vi "Read Scalar Boolean.vi"(8 "error in (no error)":errorcluster, 11 "pointer in":u64) -> (0 "error out":errorcluster, 2 "value out":bool, 3 "pointer out":u64)   [LabVIEW 2016, in "Linux RT IPC.Shared Memory.lvlib"]
uses:
  Linux RT IPC.Shared Memory.lvlib
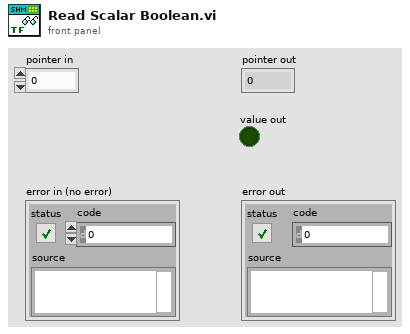
[diagram p1: front panel]
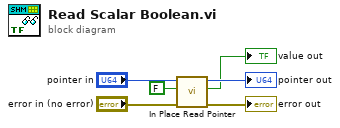
[diagram p0: block diagram]
diagram:
  n1 = call-poly "In Place Read Pointer.vi"("error in (no error)"="error in (no error)", "value in"=FALSE, "pointer in"="pointer in") -> ("error out"=→"error out":errorcluster, "value out"=→"value out":bool, "pointer out"=→"pointer out":u64)  [unwired: 6 in]
